vi "布尔值转负-引用.vi"(8 "错误输入（无错误）":errorcluster, 11 "Boolean输入":refnum<vi>) -> (0 "错误输出":errorcluster)   [LabVIEW 2017]
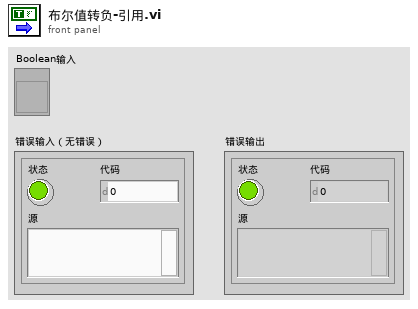
[diagram p1: front panel]
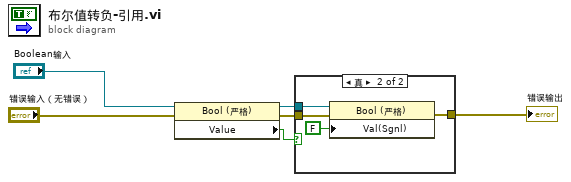
[diagram p0: block diagram]
diagram:
  n1 = property class="Bool (严格)"(reference="Boolean输入", error in="错误输入（无错误）") -> (reference out=w2:refnum<vi>, error out=w5:errorcluster, "Value"=w3:bool)
  n2 = case shown="真" w3 {
    tunnel: w2 -> [_ w11]
    tunnel: w5 -> [w7 w9]
    tunnel: [w7 w8] -> w6
    frame False {
    }
    frame True {
      n3 = property class="Bool (严格)"(reference=w11, error in=w9, "Val(Sgnl)"=FALSE ("值(信号)")) -> (error out=w8:errorcluster)  [unwired: 1 out]
    }
  }
  "错误输出" <- w6
